vi "Tag Engine_general.utest.vi"() -> ()   [LabVIEW 2020]
doc: "_Test_"
uses:
  Tag/Tag.lvclass/Tag.ctl
  Tag/Tag.lvclass
  3d4b882a-e436-4f37-aed9-35a305ddb346.vi
  eb00c9cd-5161-4d26-ae32-490fe508d5fe.vi
  73cf2a16-35a3-43c1-b628-a6dee5632637.vi
  77c790be-6133-48fa-abcc-627f330f8da1.vi
  0c08567f-0fa1-42bb-8d57-fa012ad98f57.vi
  8b0f5b2c-ae71-4c49-821c-81fbe44761c9.vi
  42aa8062-1980-4d59-a8f6-0165d054f103.vi
  437add60-3501-4199-a226-20a01a6dbd58.vi
  04bba0b0-ef6c-4016-8dc9-69a078e3e674.vi
  eaf49da9-90dd-481e-aa33-508926ab192f.vi
  Tag/Read Name.vi
  Tag/Read LockList.vi
  Tag/Read Locked.vi
  2632e44f-fe09-471c-86ff-43449fcdd828.vi
  b85cf2bc-4034-48fe-9f60-d00c2b090f68.vi
  Tag/Construct.vi
  API/Write Tag Value_ByRef.vi
  API/Get Tag.vi
  API/Get Tag Value_ByRef.vi
  Tools/SubVIs/Array of VData to VCluster_openG.vi
  Tag/Read SetRequest Event.vi
  API/Send Tag SetRequest_ByRef.vi
  Tag/Write Value with Timestamp.vi
  Tag/Read Value.vi
  Tag/Read Timestamp.vi
  Tag/Write SetRequest.vi
  Core/Get Delimiter.vi
  <vilib>/Utility/error.llb/Error Cluster From Error Code.vi
  Tag/Set Properties from Initial.vi
  Core/Add Tag.vi
  <vilib>/addons/_JKI Toolkits/Caraya/classes/Assert/Assert Not Error.vi
  Core/Tag Lookup_By Name.vi
  <vilib>/addons/_JKI Toolkits/Caraya/classes/Assert/Assert Equal Value_Variant.vi
  <vilib>/addons/_JKI Toolkits/Caraya/classes/Assert/Assert True.vi
  <vilib>/Utility/Data Type/Get Type Information.vi
  <vilib>/Utility/Data Type/Get Cluster Information.vi
  <vilib>/addons/_JKI Toolkits/Caraya/classes/Assert/Assert Error.vi
  <vilib>/addons/_JKI Toolkits/Caraya/classes/Assert/Assert False.vi
  Tag Engine.lvlib
  <vilib>/addons/_JKI Toolkits/Caraya/classes/Test/Test.lvclass
  <vilib>/addons/_JKI Toolkits/Caraya/classes/Assert/Assert.lvclass
  <vilib>/JDP Science/JSONtext/JSONtext.lvlib
panel:
  out "locked tag error":errorcluster
  out "FormatString":string
  out "Value 3":dbl
  out "Timestamp":timestamp[](array[timestamp])
  out "Value":string[](array[string])
  out "Write":dbl=42.0
  out "Read":dbl[](array[numeric])
  out "Tag Names":string[](array[string])=["GROUP1:TAG1", "GROUP1:TAG2", "GROUP1:TAG3", "GROUP1:TAG4"]
  out "Read by Ref":dbl[](array[numeric])
  out "Write by Ref":dbl[](array[numeric])
  out "Write by Name":dbl[](array[numeric])
  out "Read by Name":dbl[](array[numeric])
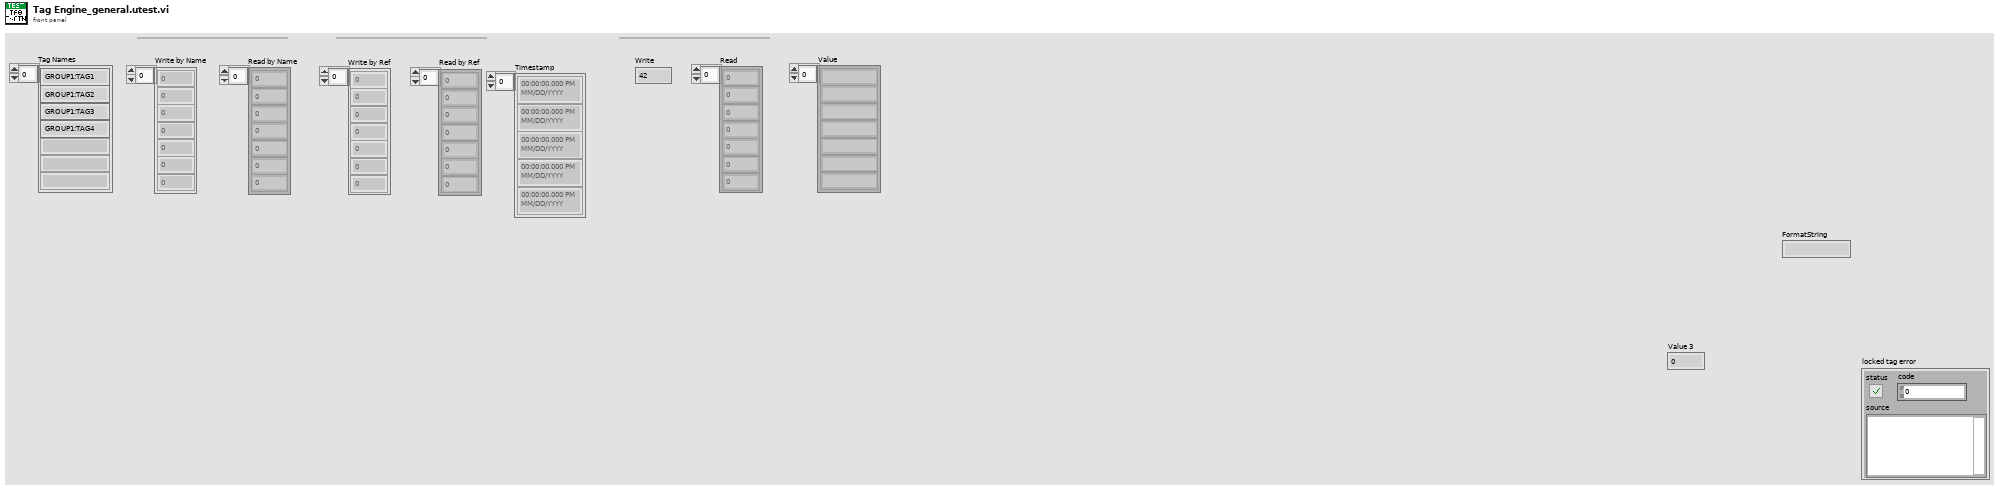
[diagram p1: front panel]
types:
  T1 = cluster{"TAG1":refnum<data-value>, "TAG2":refnum<data-value>, "TAG3":refnum<data-value>}
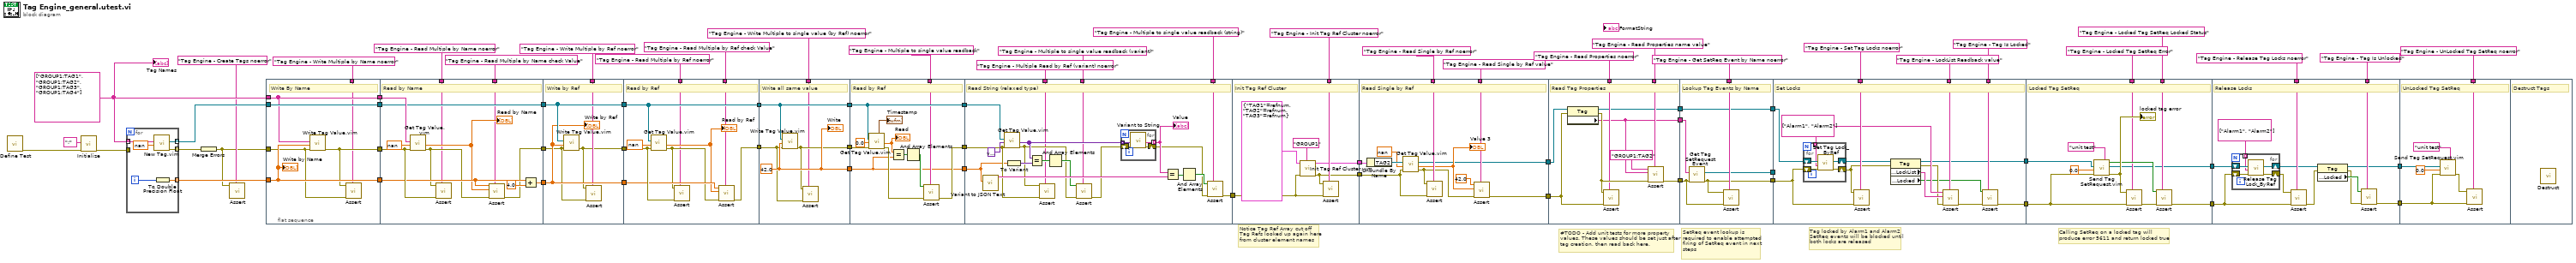
[diagram p0: block diagram]
diagram:
  w69 = string[] ["GROUP1:TAG1", "GROUP1:TAG2", "GROUP1:TAG3", "GROUP1:TAG4"]
  # "Calling SetReq on a locked tag will\nproduce error 5611 and return locked true"
  # "Tag locked by Alarm1 and Alarm2\nSetReq events will be blocked until\nboth locks are released"
  # "SetReq event lookup is\nrequired to enable attempted\nfiring of SetReq event in next\nsteps"
  # "#TODO - Add unit tests for more property\nvalues. These values should be set just after\ntag creation, then read back here."
  # "Notice Tag Ref Array cut off\nTag Refs looked up again here\nfrom cluster element names"
  n1 = call <vilib>:"Define Test.vi"() -> ("error out"=w33:errorcluster)  [unwired: 10 in, 1 out]
  n2 = call "Initialize.vi"("error in (no error)"=w33, "Namespace Delimiter"=":") -> ("error out"=w32:errorcluster)  [unwired: 9 in]
  n3 = for {
    tunnel: w69 -> [w75] mode=indexing
    tunnel: [w73] -> w53 mode=indexing
    tunnel: [w71] -> w68 mode=indexing
    tunnel: [w70] -> w52 mode=indexing
    tunnel: w32 -> [_]
    i -> [w72]
    n4 = call "New Tag.vim"("Initial Value"=nan, "Tag Name"=w75) -> ("error out"=w70:errorcluster, "Tag Ref out"=w73:refnum<data-value>)  [unwired: 8 in]
    n5 = To Double Precision Float(number=w72) -> (double precision float=w71:dbl)
  }
  n6 = Merge Errors(w52) -> (w50:errorcluster)
  n7 = call-poly <vilib>:"Assert.vi"("Label"="Tag Engine - Create Tags noerror", "Not Error?"=w50) -> ()  [unwired: 8 in, 2 out]
  n8 = flat-sequence {
    tunnel: w69 -> [w80]
    tunnel: w53 -> [w81]
    tunnel: w68 -> [w79]
    tunnel: [w80] -> w67
    tunnel: [w79] -> w66
    tunnel: [w81] -> w63
    tunnel: [w78] -> w60
    tunnel: w50 -> [w77]
    tunnel: "Tag Engine - Write Multiple by Name noerror" ("Label") -> [w76]
    tunnel: w67 -> [w93]
    tunnel: w66 -> [w87]
    tunnel: [w90] -> w65
    tunnel: [w89] -> w64
    tunnel: w63 -> [w89]
    tunnel: [w84] -> w61
    tunnel: w60 -> [w88]
    tunnel: "Tag Engine - Read Multiple by Name noerror" ("Label") -> [w83]
    tunnel: "Tag Engine - Read Multiple by Name check Value" ("Label") -> [w82]
    tunnel: w65 -> [w97]
    tunnel: w64 -> [w98]
    tunnel: [w98] -> w62
    tunnel: w61 -> [w96]
    tunnel: [w97] -> w56
    tunnel: "Tag Engine - Write Multiple by Ref noerror" ("Label") -> [w95]
    tunnel: [w94] -> w45
    tunnel: w62 -> [w106]
    tunnel: [w106] -> w59
    tunnel: w56 -> [w104]
    tunnel: w45 -> [w105]
    tunnel: [w101] -> w44
    tunnel: "Tag Engine - Read Multiple by Ref noerror" ("Label") -> [w100]
    tunnel: "Tag Engine - Read Multiple by Ref check Value" ("Label") -> [w99]
    tunnel: w59 -> [w112]
    tunnel: [w110] -> w58
    tunnel: [w112] -> w57
    tunnel: [w111] -> w55
    tunnel: w44 -> [w109]
    tunnel: "Tag Engine - Write Multiple to single value (by Ref) noerror" ("Label") -> [w108]
    tunnel: w58 -> [w123]
    tunnel: w57 -> [w119]
    tunnel: w55 -> [w113]
    tunnel: [w119] -> w54
    tunnel: "Tag Engine - Multiple to single value readback" ("Label") -> [w115]
    tunnel: [w114] -> w39
    tunnel: [w113] -> w38
    tunnel: w54 -> [w142]
    tunnel: w39 -> [w134]
    tunnel: w38 -> [w132]
    tunnel: "Tag Engine - Multiple to single value readback (string)" ("Label") -> [w136]
    tunnel: "Tag Engine - Multiple Read by Ref (variant) noerror" ("Label") -> [w126]
    tunnel: "Tag Engine - Multiple to single value readback (variant)" ("Label") -> [w125]
    tunnel: [w124] -> w31
    tunnel: w31 -> [w150]
    tunnel: "Tag Engine - Init Tag Ref Cluster noerror" ("Label") -> [w149]
    tunnel: [w148] -> w29
    tunnel: [w147] -> w28
    tunnel: w29 -> [w161]
    tunnel: w28 -> [w160]
    tunnel: "Tag Engine - Read Single by Ref noerror" ("Label") -> [w159]
    tunnel: "Tag Engine - Read Single by Ref value" ("Label") -> [w155]
    tunnel: [w154] -> w25
    tunnel: [w153] -> w24
    tunnel: w25 -> [w172]
    tunnel: w24 -> [w170]
    tunnel: "Tag Engine - Read Properties noerror" ("Label") -> [w168]
    tunnel: "Tag Engine - Read Properties name value" ("Label") -> [w167]
    tunnel: [w166] -> w21
    tunnel: [w165] -> w20
    tunnel: [w164] -> w16
    tunnel: w21 -> [w177]
    tunnel: w20 -> [w178]
    tunnel: "Tag Engine - Get SetReq Event by Name noerror" ("Label") -> [w176]
    tunnel: [w175] -> w18
    tunnel: [w174] -> w17
    tunnel: w16 -> [w174]
    tunnel: [w173] -> w15
    tunnel: w18 -> [_]
    tunnel: w17 -> [w192]
    tunnel: w15 -> [w191]
    tunnel: "Tag Engine - Set Tag Locks noerror" ("Label") -> [w190]
    tunnel: "Tag Engine - LockList Readback value" ("Label") -> [w184]
    tunnel: "Tag Engine - Tag Is Locked" ("Label") -> [w181]
    tunnel: [w180] -> w11
    tunnel: [w179] -> w10
    tunnel: w11 -> [w207]
    tunnel: w10 -> [w204]
    tunnel: "Tag Engine - Locked Tag SetReq Error" ("Label") -> [w201]
    tunnel: "Tag Engine - Locked Tag SetReq Locked Status" ("Label") -> [w200]
    tunnel: [w199] -> w7
    tunnel: [w198] -> w6
    tunnel: w7 -> [w220]
    tunnel: w6 -> [w217]
    tunnel: "Tag Engine - Release Tag Locks noerror" ("Label") -> [w216]
    tunnel: "Tag Engine - Tag Is Unlocked" ("Label") -> [w211]
    tunnel: [w210] -> w3
    tunnel: [w209] -> w2
    tunnel: w3 -> [w229]
    tunnel: w2 -> [w227]
    tunnel: "Tag Engine - UnLocked Tag SetReq noerror" ("Label") -> [w226]
    frame #0 {
      # "Write By Name"
      n9 = call "Write Tag Value.vim"("error in (no error)"=w77, "Value"=w79, "Tag Name(s)/Ref(s)"=w80) -> ("error out"=w78:errorcluster)  [unwired: 7 in, 1 out]
      n10 = call-poly <vilib>:"Assert.vi"("Label"=w76, "error in (no error)"=w77, "Not Error?"=w78) -> ()  [unwired: 7 in, 2 out]
      "Write by Name" <- w79
    }
    frame #1 {
      # "Read by Name"
      n11 = call "Get Tag Value.vim"("error in (no error)"=w88, "Default (Void)"=nan, "Tag Name(s)/Ref(s)"=w93) -> ("error out"=w85:errorcluster, "Value(s)"=w86:dbl[])  [unwired: 5 in, 2 out]
      "Read by Name" <- w86
      n12 = call-poly <vilib>:"Assert.vi"("Label"=w83, "error in (no error)"=w88, "Not Error?"=w85) -> ()  [unwired: 7 in, 2 out]
      n13 = call-poly <vilib>:"Assert.vi"("Label"=w82, "error in (no error)"=w85, "Actual"=w86, "Expected"=w87) -> ("error out"=w84:errorcluster)  [unwired: 6 in, 1 out]
      n14 = Add(x=w87, y=4.0) -> (x+y=w90:dbl[])
    }
    frame #2 {
      # "Write by Ref"
      n15 = call "Write Tag Value.vim"("error in (no error)"=w96, "Value"=w97, "Tag Name(s)/Ref(s)"=w98) -> ("error out"=w94:errorcluster)  [unwired: 7 in, 1 out]
      n16 = call-poly <vilib>:"Assert.vi"("Label"=w95, "error in (no error)"=w96, "Not Error?"=w94) -> ()  [unwired: 7 in, 2 out]
      "Write by Ref" <- w97
    }
    frame #3 {
      # "Read by Ref"
      n17 = call "Get Tag Value.vim"("error in (no error)"=w105, "Default (Void)"=nan, "Tag Name(s)/Ref(s)"=w106) -> ("error out"=w103:errorcluster, "Value(s)"=w102:dbl[])  [unwired: 5 in, 2 out]
      "Read by Ref" <- w102
      n18 = call-poly <vilib>:"Assert.vi"("Label"=w100, "error in (no error)"=w105, "Not Error?"=w103) -> ()  [unwired: 7 in, 2 out]
      n19 = call-poly <vilib>:"Assert.vi"("Label"=w99, "error in (no error)"=w103, "Actual"=w102, "Expected"=w104) -> ("error out"=w101:errorcluster)  [unwired: 6 in, 1 out]
    }
    frame #4 {
      w111 = 42.0
      # "Write all same value"
      n20 = call "Write Tag Value.vim"("error in (no error)"=w109, "Value"=w111, "Tag Name(s)/Ref(s)"=w112) -> ("error out"=w110:errorcluster)  [unwired: 7 in, 1 out]
      n21 = call-poly <vilib>:"Assert.vi"("Label"=w108, "error in (no error)"=w109, "Not Error?"=w110) -> ()  [unwired: 7 in, 2 out]
      "Write" <- w111
    }
    frame #5 {
      # "Read by Ref"
      n22 = call "Get Tag Value.vim"("error in (no error)"=w123, "Default (Void)"=0.0, "Tag Name(s)/Ref(s)"=w119) -> ("error out"=w116:errorcluster, "Value(s)"=w121:dbl[], "Timestamp(s)"=→"Timestamp":timestamp[])  [unwired: 5 in, 1 out]
      "Read" <- w121
      n23 = Equal?(x=w121, y=w113) -> (x = y?=w120:bool[])
      n24 = And Array Elements(Boolean array=w120) -> (logical AND=w117:bool)
      n25 = call-poly <vilib>:"Assert.vi"("Label"=w115, "error in (no error)"=w116, "True?"=w117) -> ("error out"=w114:errorcluster)  [unwired: 7 in, 1 out]
    }
    frame #6 {
      # "Read String (relaxed type)"
      n26 = call <vilib>:"Variant to JSON Text.vi"("Variant"=w132) -> ("<JSON>"=w139:string)  [unwired: 8 in, 2 out]
      n27 = call "Get Tag Value.vim"("error in (no error)"=w134, "Default (Void)"=variant, "Tag Name(s)/Ref(s)"=w142) -> ("error out"=w128:errorcluster, "Value(s)"=w133:variant[])  [unwired: 5 in, 2 out]
      n28 = To Variant(anything=w132) -> (Variant=w131:variant)
      n29 = Equal?(x=w133, y=w131) -> (x = y?=w130:bool[])
      n30 = call-poly <vilib>:"Assert.vi"("Label"=w126, "error in (no error)"=w134, "Not Error?"=w128) -> ()  [unwired: 7 in, 2 out]
      n31 = And Array Elements(Boolean array=w130) -> (logical AND=w129:bool)
      n32 = call-poly <vilib>:"Assert.vi"("Label"=w125, "error in (no error)"=w128, "True?"=w129) -> ("error out"=w127:errorcluster)  [unwired: 7 in, 1 out]
      n33 = for {
        tunnel: w133 -> [w146] mode=indexing
        tunnel: [w145] -> w140 mode=indexing
        shift-right: [w143] -> w135
        shift-left: w127 -> [w144]
        n34 = call "Variant to String.vi"("error in"=w144, "Variant Value"=w146) -> ("error out"=w143:errorcluster, "String Value"=w145:string)  [unwired: 8 in]
      }
      "Value" <- w140
      n35 = Equal?(x=w140, y=w139) -> (x = y?=w138:bool[])
      n36 = And Array Elements(Boolean array=w138) -> (logical AND=w137:bool)
      n37 = call-poly <vilib>:"Assert.vi"("Label"=w136, "error in (no error)"=w135, "True?"=w137) -> ("error out"=w124:errorcluster)  [unwired: 7 in, 1 out]
    }
    frame #7 {
      # "Init Tag Ref Cluster"
      n38 = call "Init Tag Ref Cluster.vim"("Namespace"="GROUP1", "error in (no error)"=w150, "Tag Refs in"=T1 {"TAG1"=refnum, "TAG2"=refnum, "TAG3"=refnum}) -> ("error out"=w147:errorcluster, "Tag Refs out"=w148:T1)  [unwired: 6 in, 1 out]
      n39 = call-poly <vilib>:"Assert.vi"("Label"=w149, "error in (no error)"=w150, "Not Error?"=w147) -> ()  [unwired: 7 in, 2 out]
    }
    frame #8 {
      # "Read Single by Ref"
      n40 = Unbundle By Name(w161) -> ("TAG2"=w163:refnum<data-value>)
      n41 = call "Get Tag Value.vim"("error in (no error)"=w160, "Default (Void)"=nan, "Tag Name(s)/Ref(s)"=w163) -> ("error out"=w156:errorcluster, "Value(s)"=w158:dbl, "Tag Ref(s) out"=w154:refnum<data-value>)  [unwired: 5 in, 1 out]
      "Value 3" <- w158
      n42 = call-poly <vilib>:"Assert.vi"("Label"=w159, "error in (no error)"=w160, "Not Error?"=w156) -> ()  [unwired: 7 in, 2 out]
      n43 = call-poly <vilib>:"Assert.vi"("Label"=w155, "error in (no error)"=w156, "Actual"=w158, "Expected"=42.0) -> ("error out"=w153:errorcluster)  [unwired: 6 in, 1 out]
    }
    frame #9 {
      # "Read Tag Properties"
      n44 = property class="Tag"(reference=w172, error in=w170) -> (reference out=w164:refnum<data-value>, error out=w169:errorcluster, "Properties:Name"=w165:string)
      n45 = call-poly <vilib>:"Assert.vi"("Label"=w168, "error in (no error)"=w170, "Not Error?"=w169) -> ()  [unwired: 7 in, 2 out]
      n46 = call-poly <vilib>:"Assert.vi"("Label"=w167, "error in (no error)"=w169, "Actual"=w165, "Expected"="GROUP1:TAG2") -> ("error out"=w166:errorcluster)  [unwired: 6 in, 1 out]
    }
    frame #10 {
      # "Lookup Tag Events by Name"
      n47 = call "Get Tag SetRequest Event.vi"("error in (no error)"=w177, "Tag Name"=w178) -> ("error out"=w173:errorcluster, "SetRequest"=w175:refnum<user-event>)  [unwired: 8 in]
      n48 = call-poly <vilib>:"Assert.vi"("Label"=w176, "error in (no error)"=w177, "Not Error?"=w173) -> ()  [unwired: 7 in, 2 out]
    }
    frame #11 {
      w186 = string[] ["Alarm1", "Alarm2"]
      # "Set Locks"
      n49 = for {
        tunnel: w186 -> [w196] mode=indexing
        shift-right: [w194] -> w188
        shift-left: w191 -> [w195]
        shift-right: [w193] -> w189
        shift-left: w192 -> [w197]
        n50 = call "Set Tag Lock_ByRef.vi"("error in (no error)"=w195, "LockName"=w196, "Tag Ref in"=w197) -> ("error out"=w194:errorcluster, "Tag Ref out"=w193:refnum<data-value>)  [unwired: 7 in]
      }
      n51 = call-poly <vilib>:"Assert.vi"("Label"=w190, "error in (no error)"=w191, "Not Error?"=w188) -> ()  [unwired: 7 in, 2 out]
      n52 = property class="Tag"(reference=w189, error in=w188) -> (reference out=w180:refnum<data-value>, error out=w185:errorcluster, "Properties:LockList"=w187:string[], "Properties:Locked"=w182:bool)
      n53 = call-poly <vilib>:"Assert.vi"("Label"=w184, "error in (no error)"=w185, "Actual"=w187, "Expected"=w186) -> ("error out"=w183:errorcluster)  [unwired: 6 in, 1 out]
      n54 = call-poly <vilib>:"Assert.vi"("Label"=w181, "error in (no error)"=w183, "True?"=w182) -> ("error out"=w179:errorcluster)  [unwired: 7 in, 1 out]
    }
    frame #12 {
      # "Locked Tag SetReq"
      n55 = call "Send Tag SetRequest.vim"("Source (anonymous)"="unit test", "error in (no error)"=w204, "Value"=0.0, "Tag Name(s)/Ref(s)"=w207) -> ("error out"=w205:errorcluster, "Tag Ref out"=w199:refnum<data-value>, "locked?"=w202:bool)  [unwired: 4 in, 1 out]
      "locked tag error" <- w205
      n56 = call-poly <vilib>:"Assert.vi"("Label"=w201, "error in (no error)"=w204, "Error?"=w205) -> ("error out"=w203:errorcluster)  [unwired: 7 in, 1 out]
      n57 = call-poly <vilib>:"Assert.vi"("Label"=w200, "error in (no error)"=w203, "True?"=w202) -> ("error out"=w198:errorcluster)  [unwired: 7 in, 1 out]
    }
    frame #13 {
      # "Release Locks"
      n58 = for {
        tunnel: string[] ["Alarm1", "Alarm2"] -> [w223] mode=indexing
        shift-right: [w222] -> w215
        shift-left: w220 -> [w225]
        shift-right: [w221] -> w218
        shift-left: w217 -> [w224]
        n59 = call "Release Tag Lock_ByRef.vi"("error in (no error)"=w224, "LockName"=w223, "Tag Ref in"=w225) -> ("error out"=w221:errorcluster, "Tag Ref out"=w222:refnum<data-value>)  [unwired: 7 in]
      }
      n60 = call-poly <vilib>:"Assert.vi"("Label"=w216, "error in (no error)"=w217, "Not Error?"=w218) -> ("error out"=w212:errorcluster)  [unwired: 7 in, 1 out]
      n61 = property class="Tag"(reference=w215, error in=w212) -> (reference out=w210:refnum<data-value>, error out=w213:errorcluster, "Properties:Locked"=w214:bool)
      n62 = call-poly <vilib>:"Assert.vi"("Label"=w211, "error in (no error)"=w213, "False?"=w214) -> ("error out"=w209:errorcluster)  [unwired: 7 in, 1 out]
    }
    frame #14 {
      # "UnLocked Tag SetReq"
      n63 = call "Send Tag SetRequest.vim"("Source (anonymous)"="unit test", "error in (no error)"=w227, "Value"=0.0, "Tag Name(s)/Ref(s)"=w229) -> ("error out"=w228:errorcluster)  [unwired: 4 in, 3 out]
      n64 = call-poly <vilib>:"Assert.vi"("Label"=w226, "error in (no error)"=w227, "Not Error?"=w228) -> ()  [unwired: 7 in, 2 out]
    }
    frame #15 {
      # "Destruct Tags"
      n65 = call "Destruct.vi"() -> ()  [unwired: 11 in, 1 out]
    }
  }
  "Tag Names" <- w69
